vi "Negotiate Protocol Version.vi"(8 "error in":errorcluster, 10 "message json":string, 11 "response":string) -> (0 "error out":errorcluster, 3 "response out":string)   [LabVIEW 2020, in "MCP Server.lvlib"]
doc: "Version negotiation of initialize.\n\nIf the client asks for a protocol version this server supports, the response answers with that version. Otherwise it answers with the first entry of Supported Protocol Versions.vi, the newest version the server supports. The choice is made by Choose Protocol Version.vi.\n\nThe list of versions is kept only in Supported Protocol Versions.vi. Validate HTTP Request.vi checks the MCP-Protocol-Version header against the same list."
uses:
  MCP Server.lvlib
  <vilib>/JDP Science/JSONtext/JSONtext.lvlib
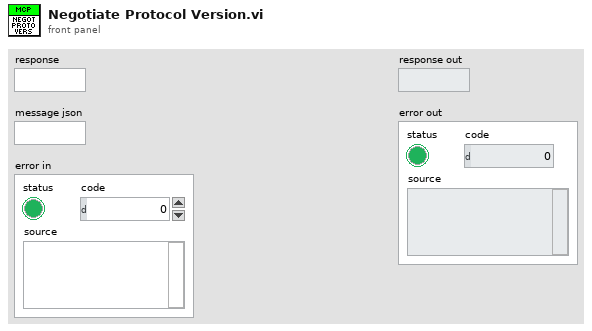
[diagram p1: front panel]
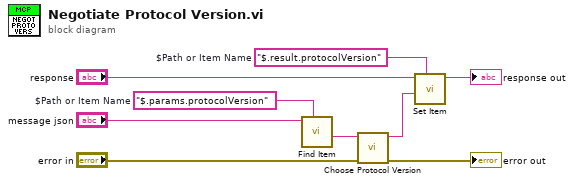
[diagram p0: block diagram]
diagram:
  w7 = "$.result.protocolVersion"  # $Path or Item Name
  w8 = "$.params.protocolVersion"  # $Path or Item Name
  n1 = call <vilib>:"Find Item.vi"("$Path or Item Name"=w8, "JSON"="message json") -> ("<JSON>"=w4:string)  [unwired: 6 in, 3 out]
  n2 = call "Choose Protocol Version.vi"("error in"="error in", "requested version"=w4) -> ("error out"=→"error out":errorcluster, "protocol version"=w3:string)  [unwired: 8 in]
  n3 = call <vilib>:"Set Item.vi"("$Path or Item Name"=w7, "JSON to Insert"=w3, "JSON"="response") -> ("<JSON>"=→"response out":string)  [unwired: 5 in, 2 out]
